vi "PicoScope3000aExampleRapidBlockBulkMSO.vi"() -> ()   [LabVIEW 2009]
uses:
  <vilib>/Waveform/DWDTOps.llb/DWDT Analog to Digital.vi
panel:
  in  "Trigger Conditions":T1 {"Condition Logic" items=["AND", "OR", "XOR"]}
  in  "Digital Port  0":T2 {"Direction Channel 7" items=["Don't Care", "Low", "High", "Rising", "Falling"]; "Direction Channel 6" items=["Don't Care", "Low", "High", "Rising", "Falling"]; "Direction Channel 5" items=["Don't Care", "Low", "High", "Rising", "Falling"]; "Direction Channel 4" items=["Don't Care", "Low", "High", "Rising", "Falling"]; "Direction Channel 3" items=["Don't Care", "Low", "High", "Rising", "Falling"]; "Direction Channel 2" items=["Don't Care", "Low", "High", "Rising", "Falling"]; "Direction Channel 1" items=["Don't Care", "Low", "High", "Rising", "Falling"]; "Direction Channel 0" items=["Don't Care", "Low", "High", "Rising", "Falling"]}
  out "Port 0 Digital Waveform Graph":digitalwaveform(graph)
  in  "Port 0 Settings":cluster{"Enabled":bool, "Logic Level":u16} {"Logic Level" items=["1.5V TTL", "2.5V CMOS"]}
  in  "MSO Device?":bool
  in  "Trigger Settings":T3 {"Trigger Direction" items=["Rising", "Falling"]}
  in  "Channel A Settings":T4 {"Range" items=["10 mV", "20 mV", "50 mV", "100 mV", "200 mV", "500 mV", "1 V", "2 V", "5 V", "10 V", "20 V", "50 V ", "100 V"]; "Coupling" items=["AC", "DC"]}
  in  "Rapid Block Acquisition Settings":T5
  out "Capture Complete":bool
  in  "Run":bool
  out "Channel A":i16[](graph)
  in  "Capture Index":i16 min=0
  in  "stop":bool
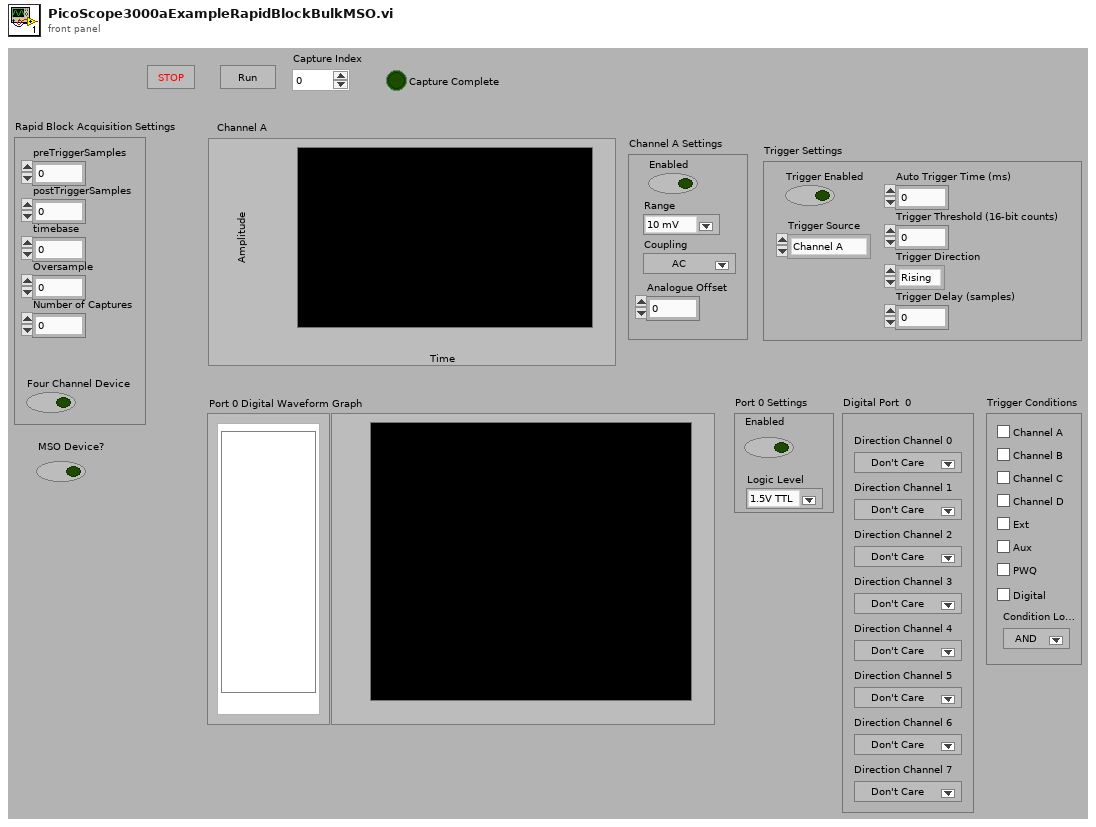
[diagram p1: front panel]
types:
  T1 = cluster{"Channel A":bool, "Channel B":bool, "Channel C":bool, "Channel D":bool, "Aux":bool, "PWQ":bool, "Condition Logic":u16, "Ext":bool, "Digital":bool}
  T2 = cluster{"Direction Channel 0":u16, "Direction Channel 1":u16, "Direction Channel 2":u16, "Direction Channel 3":u16, "Direction Channel 4":u16, "Direction Channel 5":u16, "Direction Channel 6":u16, "Direction Channel 7":u16}
  T3 = cluster{"Trigger Enabled":bool, "Trigger Source":enum16{"Channel A", "Channel B", "Channel C", "Channel D", "Ext."}, "Trigger Threshold (16-bit counts)":i16, "Trigger Direction":u16, "Trigger Delay (samples)":u32, "Auto Trigger Time (ms)":i16}
  T4 = cluster{"Enabled":bool, "Coupling":i16, "Range":u16, "Analogue Offset":sgl}
  T5 = cluster{"preTriggerSamples":u32, "postTriggerSamples":u32, "timebase":u32, "Four Channel Device":bool, "Oversample":i16, "Number of Captures":u32}
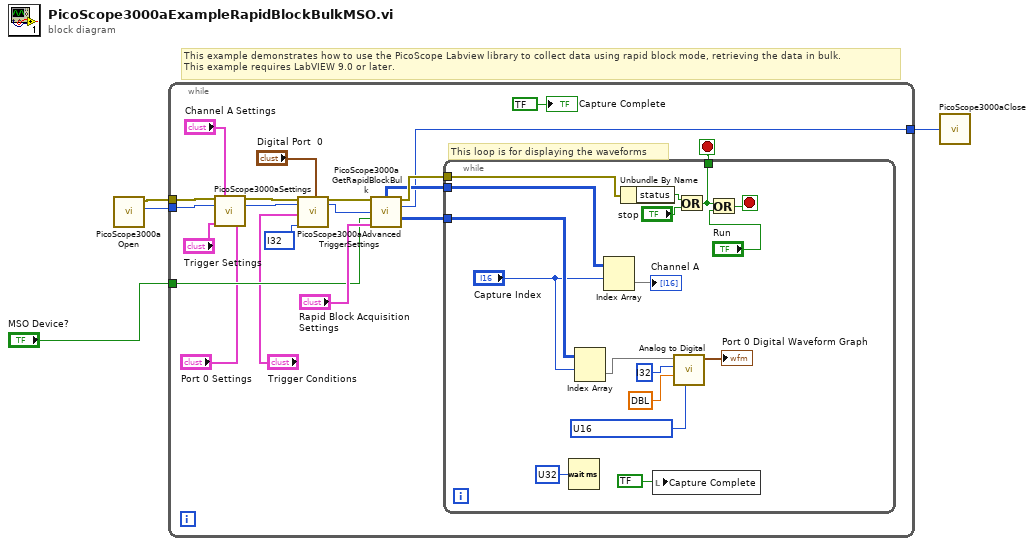
[diagram p0: block diagram]
diagram:
  # "This example demonstrates how to use the PicoScope Labview library to collect data using rapid block mode, retrieving the data in bulk.\nThis example requires LabVIEW 9.0 or later."
  n1 = call "PicoScope3000aOpen.vi"() -> ("handle"=w2:i16, "error out"=w3:errorcluster)  [unwired: 6 in, 4 out]
  n2 = while {
    tunnel: [w19] -> w4
    tunnel: w3 -> [w16]
    tunnel: w2 -> [w15]
    tunnel: "MSO Device?" -> [w14]
    stop <- w24 stop-if-true
    # "This loop is for displaying the waveforms"
    n3 = call "PicoScope3000aSettings.vi"("error in"=w16, "Channel A Settings"="Channel A Settings", "Port 0 Settings"="Port 0 Settings", "handle in"=w15, "Trigger Settings"="Trigger Settings") -> ("error out"=w9:errorcluster, "handle out"=w8:i16)  [unwired: 8 in, 1 out]
    n4 = call "PicoScope3000aAdvancedTriggerSettings.vi"("error in"=w9, "handle in"=w8, "Trigger Conditions"="Trigger Conditions", "Auto Trigger (ms)"=i32 ?, "Digital Port  0"="Digital Port  0") -> ("error out"=w11:errorcluster, "handle out"=w10:i16)  [unwired: 13 in]
    n5 = call "PicoScope3000aGetRapidBlockBulk.vi"("error in"=w11, "handle in"=w10, "MSO Device?"=w14, "Rapid Block Acquisition Settings"="Rapid Block Acquisition Settings") -> ("Channel A Buffer"=w20:i16[][], "error out"=w21:errorcluster, "handle out"=w19:i16, "Port 0 Buffer"=w12:i16[][])  [unwired: 3 in, 5 out]
    n6 = while {
      tunnel: [w40] -> w24
      tunnel: w20 -> [w26]
      tunnel: w21 -> [w35]
      tunnel: w12 -> [w29]
      stop <- w39 stop-if-true
      w30 = u16 ? items=["unsigned binary", "offset binary", "2's complement"] ("data format (offset binary)")
      n7 = Wait (ms)(milliseconds to wait=u32 ?) -> ()  [unwired: 1 out]
      n8 = Index Array(array=w29, index (row)="Capture Index") -> (element=w28:i16[])  [unwired: 1 in]
      n9 = Index Array(array=w26, index (row)="Capture Index") -> (element=→"Channel A":i16[])  [unwired: 1 in]
      n10 = Unbundle By Name(w35) -> ("status"=w34:bool)
      n11 = local write "Capture Complete"(bool ? ("Capture Complete")) -> ()
      n12 = call-poly <vilib>:"Analog to Digital.vi"("data format (offset binary)"=w30, "full-scale range (pk-pk)"=dbl ?, "resolution (16 bit)"=i32 ?, "analog waveform"=w28) -> ("digital waveform"=→"Port 0 Digital Waveform Graph":digitalwaveform)  [unwired: 4 in, 3 out]
      n13 = Or(x=w34, y="stop") -> (x .or. y?=w40:bool)
      n14 = Or(x=w40, y="Run") -> (x .or. y?=w39:bool)
    }
    "Capture Complete" <- bool ? ("Capture Complete")
  }
  n15 = call "PicoScope3000aClose.vi"("handle"=w4) -> ()
